vi "Translate text.vi"(7 "Translate? (T)":bool=TRUE, 8 "error in (no error)":errorcluster, 10 "Language(\"\"=Startup Language)":string, 11 "Constant":string) -> (0 "error out":errorcluster, 3 "Output":string)   [LabVIEW 2019, in "Language Selection.lvlib"]
doc: "Translates a string text to the input language.\n\nIf \"Translate?\" is false, the input text string will pass directly to the output.\nNB: This function does not support unicode translation.\n- - -\nCopyright (c) 2026, Merecs Engineering GmbH"
uses:
  Language Selection.lvlib
  TypeDefs/Cluster PropertyTranslation.ctl
  TypeDefs/Enum Property Type.ctl
  <vilib>/Utility/error.llb/Clear Errors.vi
  private/Set use unicode and default Lang.vi
  <vilib>/Utility/error.llb/Trim Whitespace.vi
  private/Boolean Translate.vi
  Update Controls/Update MC Listbox vColumn headers.vi
  Update Controls/Update Listbox headers.vi
  Update Controls/Tool_Unicode Update Table Headers.vi
  Update Controls/update Graph.vi
  Update Controls/update 1D array.vi
  Update Controls/update tree column header.vi
  Update Controls/update 2D array.vi
  Update Controls/update listbox Items.vi
  Update Controls/update MultiColumn Listbox Items.vi
  Update Controls/Tool_Unicode Update Table Data.vi
  Update Controls/Update caption.vi
  Update Controls/update ring.vi
  <vilib>/addons/Tools/Unicode/Property Interpret As Unicode.vi
  <vilib>/addons/Tools/Unicode/Convert ASCII to UTF-16LE.vi
  <vilib>/addons/Tools/Unicode/_subVIs/Convert ASCII to UTF-16LE (1D).vi
  Update Controls/Update String value.vi
  Update Controls/Tool_Unicode Update Tab Control Pages.vi
  packages/error-generation/src/Error Generation/Add Argument.vi
panel:
  out "Unicode?":bool
  # "Connector Pane"
  # "Locals"
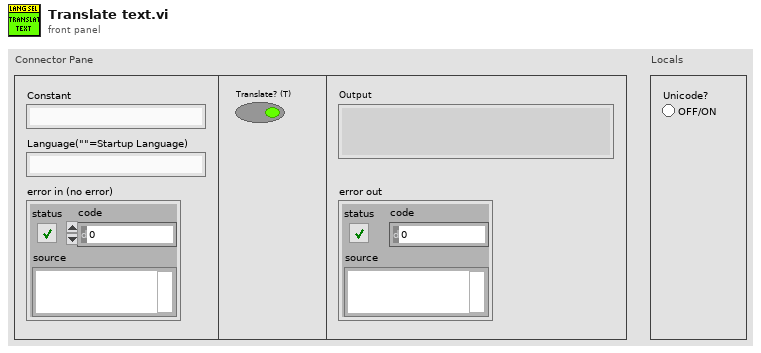
[diagram p1: front panel]
types:
  T1 = typedef "Language Selection.lvlib/Enum Property Type.ctl" = enum16{"NA", "Caption", "String Value", "Boolean Text", "Ring Strings", "1D Array Elements", "2D Array Elements", "(MC)Listbox Header", "(MC)Listbox Items", "Tab Pages Names", "X & Y GraphChart", "Plot Names", "Table Headers", "Table Items", "TipStrip", "Combobox Strings", "Cursor Name", "Tree Col Headers"}
  T2 = typedef "Language Selection.lvlib/Cluster PropertyTranslation.ctl" = cluster{"Type":T1, "Translation ANSI":string[], "Translation Unicode":string[]}
  T3 = typedef "Language Selection.lvlib/Cluster LanguageClusterWithRefnum.ctl" = cluster{"Property":T2[], "Controls":set{refnum<vi>}}
  T4 = typedef "Language Selection.lvlib/Enum Language.ctl" = i32
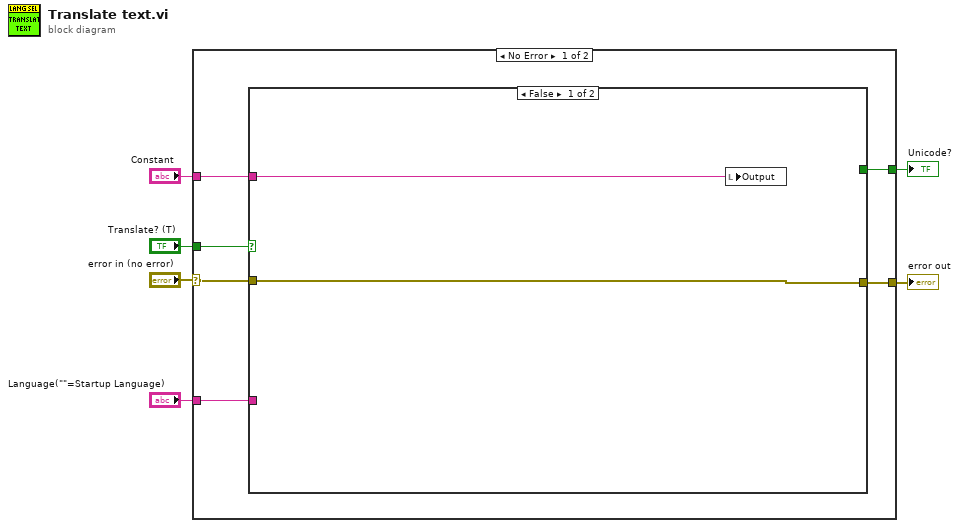
[diagram p0: block diagram]
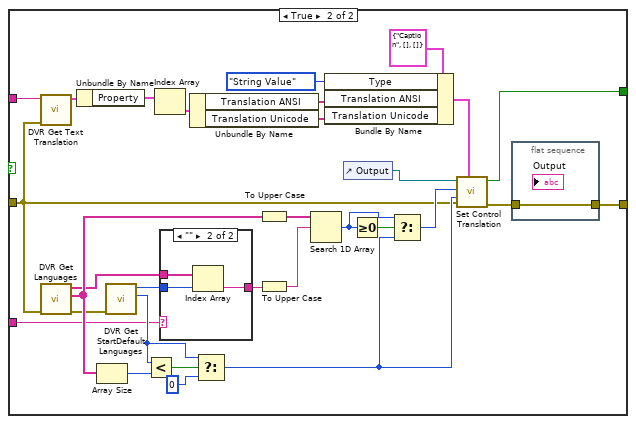
[diagram p2: hidden frame]
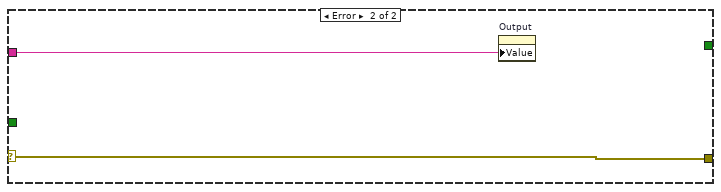
[diagram p4: hidden frame]
diagram:
  n1 = case shown="No Error" "error in (no error)" {
    selector: "error in (no error)" -> [w8 w50]
    tunnel: "Language(\"\"=Startup Language)" -> [w12 _]
    tunnel: "Constant" -> [w11 w51]
    tunnel: "Translate? (T)" -> [w10 _]
    tunnel: [w9 w50] -> w6
    tunnel: [w7 _] -> w1
    frame No Error {
      n2 = case shown="False" w10 {
        tunnel: w12 -> [_ w19]
        tunnel: w11 -> [w13 w26]
        tunnel: [w14 w20] -> w9
        tunnel: w8 -> [w14 w15]
        tunnel: [_ w32] -> w7
        frame False {
          n3 = local write "Output"(w13) -> ()
        }
        frame True {
          n4 = call "DVR Get Text Translation.vi"("error in (no error)"=w15, "Constante"=w26) -> ("Constante"=w25:T3)  [unwired: 8 in, 1 out]
          n5 = call "DVR Get Languages.vi"("error in (no error)"=w15) -> ("error out"=w18:errorcluster, "ANSI"=w44:string[], "Languages"=w24:string[])  [unwired: 7 in, 1 out]
          n6 = Unbundle By Name(w25) -> ("Property"=w37:T2[])
          n7 = Array Size(array=w44) -> (size(s)=w31:i32)
          n8 = call "DVR Get StartDefault Languages.vi"("error in (no error)"=w18) -> ("Default"=w22:i32, "Start"=w23:T4)  [unwired: 8 in, 1 out]
          n9 = Less?(x=w22, y=w31) -> (x < y?=w30:bool)
          n10 = Index Array(array=w37) -> (element=w38:T2)  [unwired: 1 in]
          n11 = case shown="\"\"" w19 {
            selector: w19 -> [w46 _]
            tunnel: [w46 w48] -> w27
            tunnel: w24 -> [_ w49]
            tunnel: w23 -> [_ w47]
            frame Default {
            }
            frame "" {
              n12 = Index Array(array=w49, index=w47) -> (element=w48:string)
            }
          }
          n13 = Unbundle By Name(w38) -> ("Translation ANSI"=w40:string[], "Translation Unicode"=w41:string[])
          n14 = Select(t=w22, s=w30, f=0 ("index")) -> (s? t:f=w17:i32)
          n15 = To Upper Case(1:w44) -> (0:w35:string[])
          n16 = To Upper Case(1:w27) -> (0:w36:string)
          n17 = Search 1D Array(1D array=w35, element=w36) -> (index of element=w16:i32)  [unwired: 1 in]
          n18 = Bundle By Name(cluster=T2 {"Type"=enum."Caption", "Translation ANSI"=[], "Translation Unicode"=[]} ("Obj."), "Type"=Enum_Property_Type."String Value", "Translation ANSI"=w40, "Translation Unicode"=w41) -> (w42:T2)
          n19 = control-ref of="Output"() -> (w43:refnum<vi>)
          n20 = Greater Or Equal To 0?(x=w16) -> (x >= 0?=w34:bool)
          n21 = Select(t=w16, s=w34, f=w17) -> (s? t:f=w33:i32)
          n22 = call "Set Control Translation.vi"("Obj."=w42, "error in (no error)"=w15, "Default Lang"=w17, "Language"=w33, "Control in"=w43) -> ("error out"=w21:errorcluster, "Unicode?"=w32:bool)  [unwired: 5 in]
          n23 = flat-sequence {
            tunnel: [w45] -> w20
            tunnel: w21 -> [w45]
            frame #0 {
            }
          }
        }
      }
    }
    frame Error {
      n24 = property on="Output" class="Str"("Value"=w51) -> ()  [unwired: 2 in, 2 out]
    }
  }
  "error out" <- w6
  "Unicode?" <- w1
